vi "Latency Reader.vi"(11 "plugin gRPC address":string="localhost:51930") -> ()   [LabVIEW 2021, in "CAN_Reader_CANsub_Test_Helpers.lvlib"]
doc: "Latency test receiver for the CAN reader plugin. For each frame: writer path = bus time - T_Out, reader path = T0 - bus time, full loop = T0 - T_Out (T_Out from the payload, bus time from the pcap packet, T0 from the FIFO header). Writes counts, statistics and 10 us histograms to a text file at the stop."
uses:
  CAN_Reader_CANsub_Test_Helpers.lvlib
  <vilib>/CIF Foundation/CIF Core/CIFCore/Class/CIFCorePlugin.lvclass/CIFCorePlugin.ctl
  <vilib>/CIF Foundation/CIF Utilities/Statistics/I64/Stats_I64_CIF_U.lvclass/Stats_I64_CIF_U.ctl
  <vilib>/CIF Foundation/CIF XNET CAN RW/XNET CAN RW.lvclass
  <vilib>/CIF Foundation/CIF Channels Core/CIFChannels/CIFChannels.lvclass
  <vilib>/CIF Foundation/CIF Core/CIFCore/Grpc/CIFCoreWrapper/CIFCoreWrapper.lvlib
  <vilib>/CIF Foundation/CIF Core/CIFCore/Class/CIFCorePlugin.lvclass
  Common/Typedef/Channels.ctl
  Common/CAN_Reader_CANsub_Common.lvlib
  Grpc/CAN_Reader_CANsub_wrapper/CAN_Reader_CANsub_Wrapper.lvlib
  <vilib>/CIF Foundation/CIF Utilities/Time/Time_CIF_U.lvlib
  <vilib>/CIF Foundation/CIF Core/CIFCore/Common/Typedef/Plugin State.ctl
  <vilib>/CIF Foundation/CIF Core/CIFCore/common/CIFCoreCommon.lvlib
  <vilib>/CIF Foundation/CIF Core/CIFCore/Common/Typedef/Timing Stats Base.ctl
  <vilib>/CIF Foundation/CIF Core/CIFCore/Common/Typedef/Timing Statistics.ctl
  <vilib>/CIF Foundation/CIF Core/CIFCore/Common/Typedef/FIFO Statistics.ctl
  <vilib>/CIF Foundation/CIF Core/CIFCore/Common/Typedef/Simple Error.ctl
  <vilib>/CIF Foundation/CIF Core/CIFCore/Common/Typedef/Monitor Doubles.ctl
  <vilib>/CIF Foundation/CIF Core/CIFCore/Common/Typedef/Monitor U64.ctl
  <vilib>/CIF Foundation/CIF Core/CIFCore/Common/Typedef/Monitor I64.ctl
  <vilib>/CIF Foundation/CIF Core/CIFCore/Common/Typedef/gRPC Reported Plugin Status.ctl
  <vilib>/CIF Foundation/CIF Channels Core/ChannelCommon/typedef/FIFO Header.ctl
  <vilib>/CIF Foundation/CIF Channels Core/ChannelCommon/ChannelCommon.lvlib
  <vilib>/xnet/xnet.llb/XNET Frame Type CAN.ctl
  <vilib>/xnet/xnet.llb/XNET Frame CAN.ctl
  Latency/Latency Metric.ctl
panel:
  out "file":path
  out "frames":u32
  out "full loop":T1
  out "reader path":T1
  out "writer path":T1
  in  "clock correction (ns)":i64=37000000000
  out "Raw Bytes":string
  out "XNET CAN Data":T2[](array[typedef]) {"payload" format="%x"; "timestamp" format="%<%.7X\n%x>T"; "type" items=["CAN Data"=0, "CAN Remote"=1, "CAN Bus Error"=2, "CAN 2.0 Data"=8, "CAN FD Data"=16, "CAN FD+BRS Data"=24, "J1939 Data"=192, "Delay"=224, "Log Trigger"=225, "Start Trigger"=226]; "identifier" format="%x"}
  out "Header":T4
  out "Node Status":T5 {"Monitor Doubles"."4" format="%#_9g"; "Monitor Doubles"."3" format="%#_9g"; "Monitor Doubles"."2" format="%#_9g"; "Monitor Doubles"."1" format="%#_9g"; "Timing Statistics (us)"."Period"."Avg" format="%_6g"}
  in  "EXIT":bool
  in  "Unload":bool
  out "error out":errorcluster
  # "Update plugin gRPC address including gRPC port and run on same target as the plugin code. \nExit will stop this VI.\nUnload will stop this VI and unload the plugin."
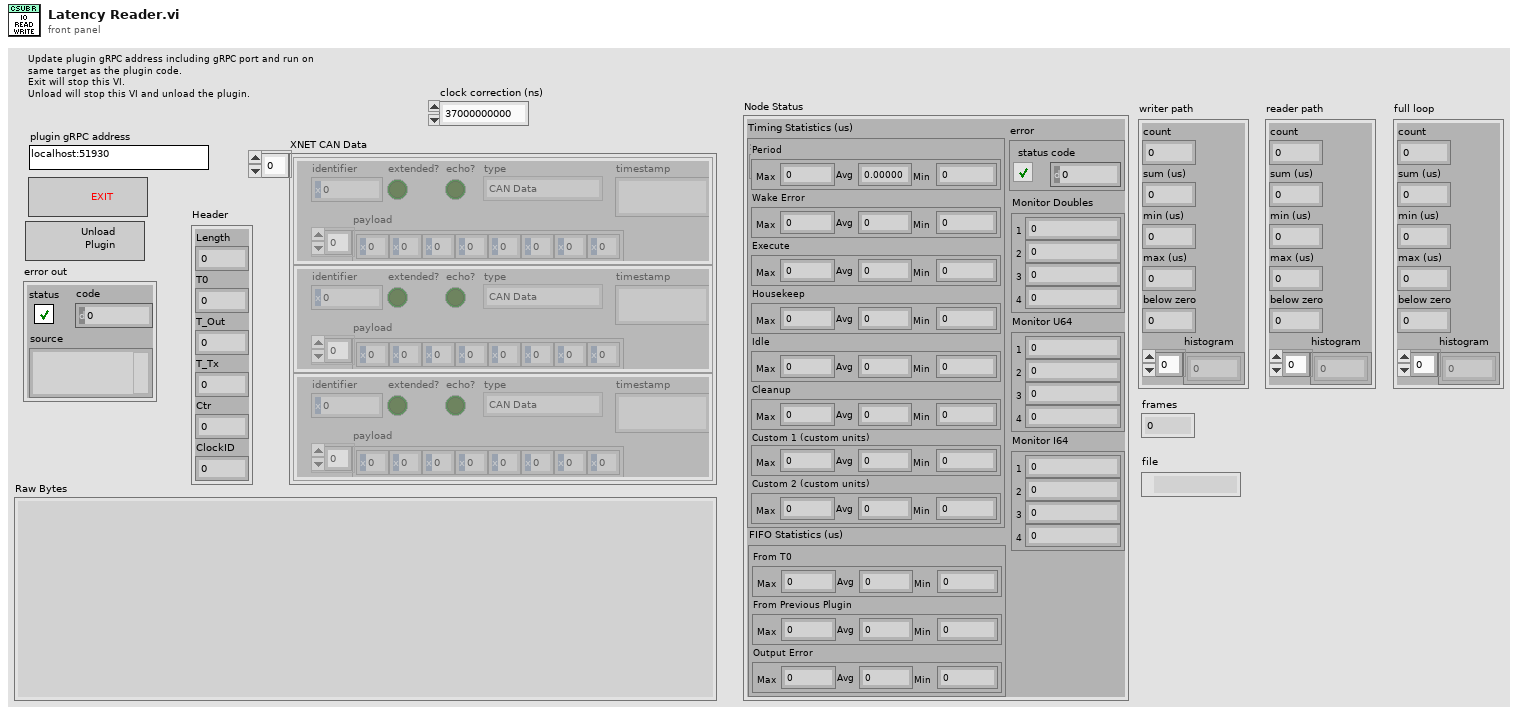
[diagram p1: front panel]
types:
  T1 = typedef "CAN_Reader_CANsub_Test_Helpers.lvlib/Latency Metric.ctl" = cluster{"count":u32, "sum (us)":dbl, "min (us)":dbl, "max (us)":dbl, "below zero":u32, "histogram":u32[]}
  T2 = typedef "XNET Frame CAN.ctl" = cluster{"timestamp":timestamp, "payload":u8[], "identifier":u32, "type":T3, "extended?":bool, "echo?":bool}
  T3 = typedef "XNET Frame Type CAN.ctl" = u8
  T4 = typedef "ChannelCommon.lvlib/FIFO Header.ctl" = cluster{"Length":u64, "T0":i64, "T_Out":i64, "T_Tx":i64, "Ctr":u64, "ClockID":u8}
  T5 = typedef "CIFCoreCommon.lvlib/gRPC Reported Plugin Status.ctl" = cluster{"State":T6, "Timing Statistics (us)":T7, "FIFO Statistics (us)":T9, "error":T10, "Monitor Doubles":T11, "Monitor U64":T12, "Monitor I64":T13}
  T6 = typedef "CIFCoreCommon.lvlib/Plugin State.ctl" = enum8{"Null", "Creating", "Listening", "Running", "CleaningUp", "Destroying", "Prepared", "FTE_Run"}
  T7 = typedef "CIFCoreCommon.lvlib/Timing Statistics.ctl" = cluster{"Period":T8, "Wake Error":T8, "Execute":T8, "Housekeep":T8, "Idle":T8, "Cleanup":T8, "Custom 1 (custom units)":T8, "Custom 2 (custom units)":T8}
  T8 = typedef "CIFCoreCommon.lvlib/Timing Stats Base.ctl" = cluster{"Max":i64, "Avg":dbl, "Min":i64}
  T9 = typedef "CIFCoreCommon.lvlib/FIFO Statistics.ctl" = cluster{"From T0":T8, "From Previous Plugin":T8, "Output Error":T8}
  T10 = typedef "CIFCoreCommon.lvlib/Simple Error.ctl" = cluster{"status":bool, "code":i32}
  T11 = typedef "CIFCoreCommon.lvlib/Monitor Doubles.ctl" = cluster{"1":dbl, "2":dbl, "3":dbl, "4":dbl}
  T12 = typedef "CIFCoreCommon.lvlib/Monitor U64.ctl" = cluster{"1":u64, "2":u64, "3":u64, "4":u64}
  T13 = typedef "CIFCoreCommon.lvlib/Monitor I64.ctl" = cluster{"1":i64, "2":i64, "3":i64, "4":i64}
  T14 = typedef "grpc-lvsupport-release.lvlib/grpcId.ctl" = u64
  T15 = typedef "CIFCoreChannel_client.lvlib/cif_management_common_Channel.ctl" = cluster{"name":string, "direction":T16, "type":string, "custom_config":u8[], "connected":bool, "connected_name":string, "forced":bool, "channel_pattern":T17}
  T16 = typedef "CIFCoreChannel_client.lvlib/cif_management_common_ChannelDirection.ctl" = enum32{"CHANNELDIRECTION_UNKNOWN", "CHANNELDIRECTION_PUBLISHER", "CHANNELDIRECTION_SUBSCRIBER"}
  T17 = typedef "CIFCoreChannel_client.lvlib/cif_management_common_ChannelPattern.ctl" = enum32{"CHANNELPATTERN_UNKNOWN", "CHANNELPATTERN_TAG", "CHANNELPATTERN_FIFO", "CHANNELPATTERN_MULTIFIFO", "CHANNELPATTERN_BACKPRESSUREFIFO"}
  T18 = typedef "CAN_Reader_CANsub_Common.lvlib/Channels.ctl" = enum16{"CAN_Frames"}
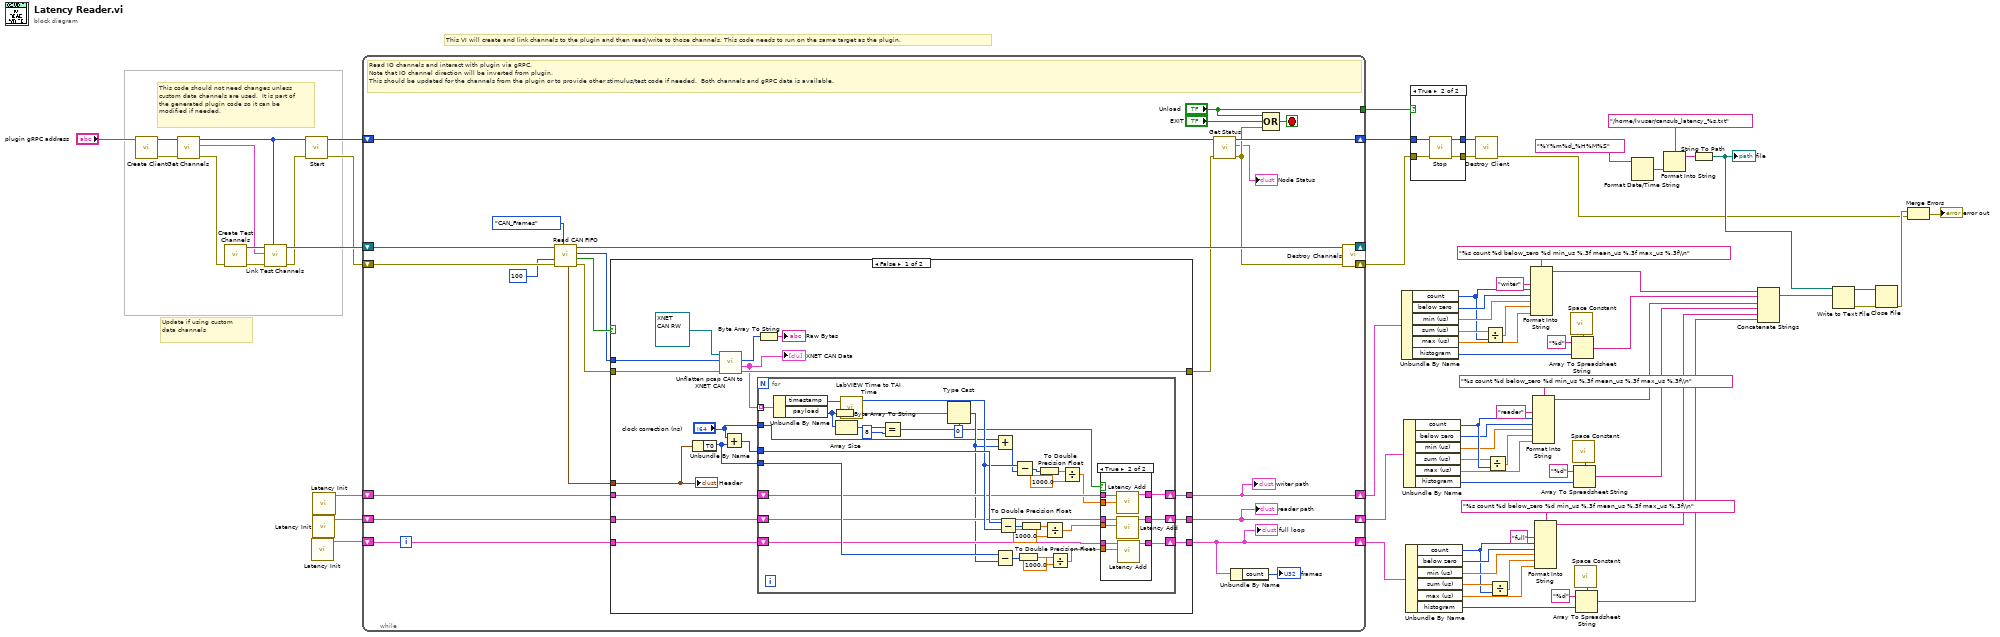
[diagram p0: block diagram]
diagram:
  # "Update if using custom data channels"
  # "This code should not need changes unless custom data channels are used.  It is part of the generated plugin code so it can be modified if needed."
  # "This VI will create and link channels to the plugin and then read/write to those channels. This code needs to run on the same target as the plugin."
  n1 = call "Create Client.vi"("address"="plugin gRPC address") -> ("error out"=w67:errorcluster, "gRPC ID Out"=w66:T14)  [unwired: 9 in]
  n2 = call <vilib>:"Get Channels.vi"("error in"=w67, "gRPC ID"=w66) -> ("error out"=w74:errorcluster, "Channels"=w70:T15[], "gRPC ID out"=w65:T14)  [unwired: 7 in]
  n3 = call "Create Test Channels.vi"("error in"=w74) -> ("error out"=w73:errorcluster, "CIFCorePlugin out"=w72:refnum<class "CIFCorePlugin.lvclass">)  [unwired: 9 in]
  n4 = call "Link Test Channels.vi"("gRPC ID in"=w65, "error in (no error)"=w73, "Channels"=w70, "CIFCorePlugin in"=w72) -> ("error out"=w63:errorcluster, "CIFCorePlugin out"=w71:refnum<class "CIFCorePlugin.lvclass">)  [unwired: 6 in]
  n5 = call <vilib>:"Start.vi"("error in"=w63, "gRPC ID"=w65) -> ("error out"=w62:errorcluster, "gRPC ID out"=w64:T14)  [unwired: 8 in]
  n6 = call "Latency Init.vi"() -> ("latency metric"=w54:T1)  [unwired: 11 in]
  n7 = call "Latency Init.vi"() -> ("latency metric"=w55:T1)  [unwired: 11 in]
  n8 = call "Latency Init.vi"() -> ("latency metric"=w56:T1)  [unwired: 11 in]
  n9 = while {
    shift-right: [w97] -> w75
    shift-left: w71 -> [w90]
    shift-right: [w96] -> w69
    shift-left: w62 -> [w89]
    shift-right: [w98] -> w60
    shift-left: w64 -> [w99]
    tunnel: ["Unload"] -> w57
    shift-right: [w79] -> w48
    shift-left: w56 -> [w82]
    shift-right: [w78] -> w16
    shift-left: w55 -> [w81]
    shift-right: [w77] -> w15
    shift-left: w54 -> [w80]
    stop <- w95 stop-if-true
    # "Read IO channels and interact with plugin via gRPC.\nNote that IO channel direction will be inverted from plugin.\nThis should be updated for the channels from the plugin or to provide other stimulus/test code if needed.  Both channels and gRPC data is available."
    n10 = call <vilib>:"Read CAN FIFO.vi"("Channel Index"=Channels."CAN_Frames" ("Channels"), "error in (no error)"=w89, "Timeout (ms)"=100, "CIFCorePlugin in"=w90) -> ("error out"=w84:errorcluster, "timed out?"=w86:bool, "Data"=w85:u8[], "CIFCorePlugin out"=w97:refnum<class "CIFCorePlugin.lvclass">, "Header"=w88:T4)  [unwired: 3 in]
    n11 = case shown="False" w86 {
      tunnel: w88 -> [w110 _]
      tunnel: w85 -> [w116 _]
      tunnel: w84 -> [w115 w164]
      tunnel: [w114 w164] -> w83
      tunnel: w82 -> [w106 w163]
      tunnel: w81 -> [w105 w162]
      tunnel: w80 -> [w104 w161]
      tunnel: [w103 w163] -> w79
      tunnel: [w102 w162] -> w78
      tunnel: [w101 w161] -> w77
      frame False {
        n12 = Unbundle By Name(w110) -> ("T0"=w107:i64)
        n13 = call <vilib>:"Unflatten pcap CAN to XNET CAN.vi"("error in (no error)"=w115, "pcap CAN DATA in"=w116, "XNET_CAN_RW in"=refnum<class "XNET CAN RW.lvclass"> refnum) -> ("error out"=w114:errorcluster, "XNET CAN Data"=w109:T2[], "pcap CAN DATA out"=w111:u8[])  [unwired: 3 in, 3 out]
        "XNET CAN Data" <- w109
        n14 = Add(x="clock correction (ns)", y=w107) -> (x+y=w108:i64)
        n15 = Byte Array To String(unsigned byte array=w111) -> (string=→"Raw Bytes":string)
        n16 = for {
          tunnel: w109 -> [w148] mode=indexing
          tunnel: w108 -> [w144]
          tunnel: w107 -> [w142]
          shift-right: [w126] -> w103
          shift-left: w106 -> [w127]
          shift-right: [w129] -> w102
          shift-left: w105 -> [w130]
          shift-right: [w131] -> w101
          shift-left: w104 -> [w133]
          tunnel: "clock correction (ns)" -> [w122]
          n17 = Unbundle By Name(w148) -> ("timestamp"=w147:timestamp, "payload"=w120:u8[])
          n18 = Byte Array To String(unsigned byte array=w120) -> (string=w145:string)
          n19 = Array Size(array=w120) -> (size(s)=w119:i32)
          n20 = call <vilib>:"LabVIEW Time to TAI Time.vi"("LabVIEW Time (s)"=w147) -> ("TAI Time (ns)"=w143:i64)  [unwired: 4 in]
          n21 = Equal?(x=w119, y=8) -> (x = y?=w117:bool)
          n22 = Type Cast(type=i64 0, x=w145) -> (*(type *) &x=w123:i64)
          n23 = Add(x=w122, y=w123) -> (x+y=w121:i64)
          n24 = Subtract(x=w142, y=w123) -> (x-y=w140:i64)
          n25 = Subtract(x=w144, y=w143) -> (x-y=w141:i64)
          n26 = Subtract(x=w143, y=w121) -> (x-y=w124:i64)
          n27 = To Double Precision Float(number=w140) -> (double precision float=w137:dbl)
          n28 = To Double Precision Float(number=w141) -> (double precision float=w138:dbl)
          n29 = To Double Precision Float(number=w124) -> (double precision float=w139:dbl)
          n30 = Divide(x=w138, y=1000.0) -> (x/y=w128:dbl)
          n31 = Divide(x=w137, y=1000.0) -> (x/y=w132:dbl)
          n32 = Divide(x=w139, y=1000.0) -> (x/y=w125:dbl)
          n33 = case shown="True" w117 {
            tunnel: w133 -> [w149 w160]
            tunnel: w132 -> [_ w159]
            tunnel: [w149 w158] -> w131
            tunnel: w130 -> [w150 w157]
            tunnel: [w150 w156] -> w129
            tunnel: w128 -> [_ w155]
            tunnel: w127 -> [w151 w154]
            tunnel: [w151 w153] -> w126
            tunnel: w125 -> [_ w152]
            frame False {
            }
            frame True {
              n34 = call "Latency Add.vi"("value (us)"=w152, "metric in"=w154) -> ("metric out"=w153:T1)  [unwired: 9 in]
              n35 = call "Latency Add.vi"("value (us)"=w155, "metric in"=w157) -> ("metric out"=w156:T1)  [unwired: 9 in]
              n36 = call "Latency Add.vi"("value (us)"=w159, "metric in"=w160) -> ("metric out"=w158:T1)  [unwired: 9 in]
            }
          }
        }
        "Header" <- w110
      }
      frame True {
      }
    }
    "writer path" <- w79
    "full loop" <- w77
    "reader path" <- w78
    n37 = call <vilib>:"Get Status.vi"("error in"=w83, "gRPC ID"=w99) -> ("error out"=w96:errorcluster, "Node Status"=→"Node Status":T5, "gRPC ID out"=w98:T14)  [unwired: 7 in]
    n38 = Unbundle By Name(w77) -> ("count"=→"frames":u32)
    n39 = Compound Arithmetic op=OR("Unload", "EXIT", w96) -> (w95:bool)
  }
  n40 = call <vilib>:"Destroy Channels.vi"("error in (no error)"=w69, "CIFCorePlugin in"=w75) -> ("error out"=w61:errorcluster)  [unwired: 7 in, 2 out]
  n41 = Unbundle By Name(w48) -> ("count"=w44:u32, "below zero"=w47:u32, "min (us)"=w46:dbl, "sum (us)"=w45:dbl, "max (us)"=w42:dbl, "histogram"=w41:u32[])
  n42 = Unbundle By Name(w16) -> ("count"=w33:u32, "below zero"=w30:u32, "min (us)"=w31:dbl, "sum (us)"=w32:dbl, "max (us)"=w35:dbl, "histogram"=w36:u32[])
  n43 = Unbundle By Name(w15) -> ("count"=w22:u32, "below zero"=w25:u32, "min (us)"=w24:dbl, "sum (us)"=w23:dbl, "max (us)"=w20:dbl, "histogram"=w19:u32[])
  n44 = case shown="True" w57 {
    tunnel: w61 -> [w165 w170]
    tunnel: w60 -> [w166 w169]
    tunnel: [w166 w168] -> w59
    tunnel: [w165 w167] -> w58
    frame False {
    }
    frame True {
      n45 = call <vilib>:"Stop.vi"("error in"=w170, "gRPC ID"=w169) -> ("error out"=w167:errorcluster, "gRPC ID out"=w168:T14)  [unwired: 8 in]
    }
  }
  n46 = call "Destroy Client.vi"("error in"=w58, "gRPC ID"=w59) -> ("error out"=w2:errorcluster)  [unwired: 9 in]
  n47 = Divide(x=w45, y=w44) -> (x/y=w43:dbl)
  n48 = Divide(x=w32, y=w33) -> (x/y=w34:dbl)
  n49 = Divide(x=w23, y=w22) -> (x/y=w21:dbl)
  n50 = Format Into String(format string="%s count %d below_zero %d min_us %.3f mean_us %.3f max_us %.3f\\n", "writer" ("input 1"), w44, w47, w46, w43, w42) -> (resulting string=w14:string)  [unwired: 2 in, 1 out]
  n51 = Format Into String(format string="%s count %d below_zero %d min_us %.3f mean_us %.3f max_us %.3f\\n", "reader" ("input 1"), w33, w30, w31, w34, w35) -> (resulting string=w12:string)  [unwired: 2 in, 1 out]
  n52 = Format Into String(format string="%s count %d below_zero %d min_us %.3f mean_us %.3f max_us %.3f\\n", "full" ("input 1"), w22, w25, w24, w21, w20) -> (resulting string=w10:string)  [unwired: 2 in, 1 out]
  n53 = call <vilib>:"Space Constant.vi"() -> ("String"=w39:string)
  n54 = Array To Spreadsheet String(delimiter (Tab)=w39, array=w41, 3:"%d" ("format string")) -> (spreadsheet string=w13:string)
  n55 = call <vilib>:"Space Constant.vi"() -> ("String"=w38:string)
  n56 = Array To Spreadsheet String(delimiter (Tab)=w38, array=w36, 3:"%d" ("format string")) -> (spreadsheet string=w11:string)
  n57 = call <vilib>:"Space Constant.vi"() -> ("String"=w17:string)
  n58 = Array To Spreadsheet String(delimiter (Tab)=w17, array=w19, 3:"%d" ("format string")) -> (spreadsheet string=w9:string)
  n59 = Format Date/Time String(time format string (%c)="%Y%m%d_%H%M%S") -> (date/time string=w52:string)  [unwired: 2 in]
  n60 = Format Into String(format string="/home/lvuser/cansub_latency_%s.txt", w52) -> (resulting string=w51:string)  [unwired: 2 in, 1 out]
  n61 = String To Path(string=w51) -> (path=w8:path)
  "file" <- w8
  n62 = Concatenate Strings(w14, w13, w12, w11, w10, w9) -> (w7:string)
  n63 = Write to Text File(file (use dialog)=w8, text=w7) -> (refnum out=w5:refnum<file>, error out=w6:errorcluster)  [unwired: 2 in, 1 out]
  n64 = Close File(refnum=w5, error in=w6) -> (error out=w3:errorcluster)  [unwired: 1 out]
  n65 = Merge Errors(w3, w2) -> (→"error out":errorcluster)
